vi "load vi modification tools.vi"() -> ()   [LabVIEW 2013, in "vi mod UI.lvlib"]
uses:
  vi mod UI.lvlib
  VI modification.lvclass
  collection/VI modification collection.lvclass
  collection/VI modification collection.lvclass/VI modification collection.ctl
  collection/Read current file list.vi
panel:
  in  "Report":i32(listbox)
  in  "Remove path":bool
  in  "add search":bool
  in  "Paths":i32(listbox)
  in  "run":bool
  in  "remove mod":bool
  in  "add mod":bool
  in  "Selected Tools":i32(listbox)
  in  "Available Tools":i32(listbox)
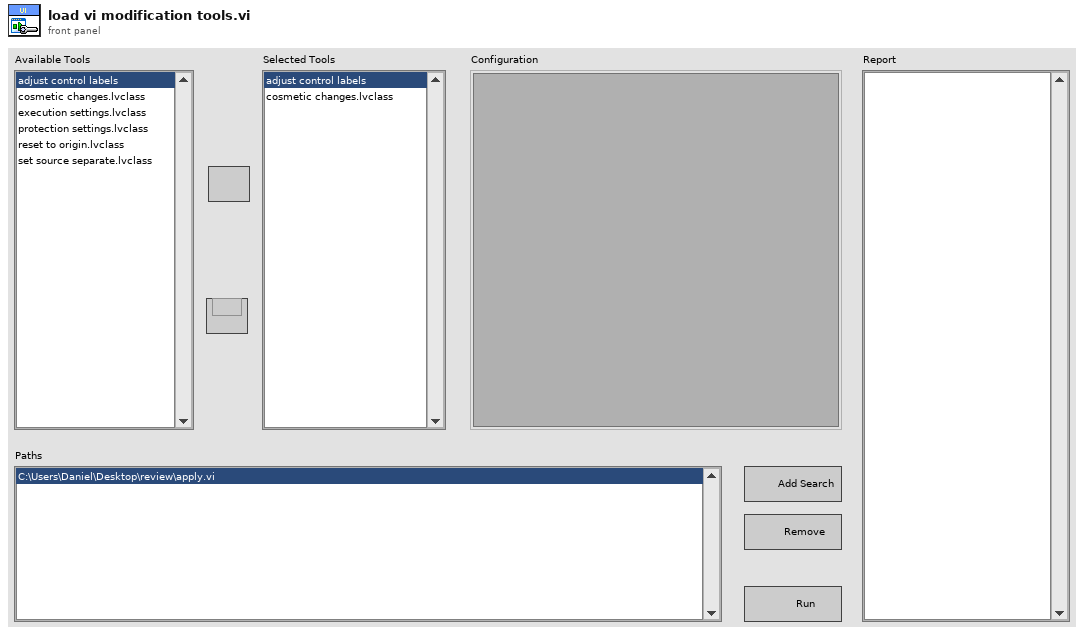
[diagram p1: front panel]
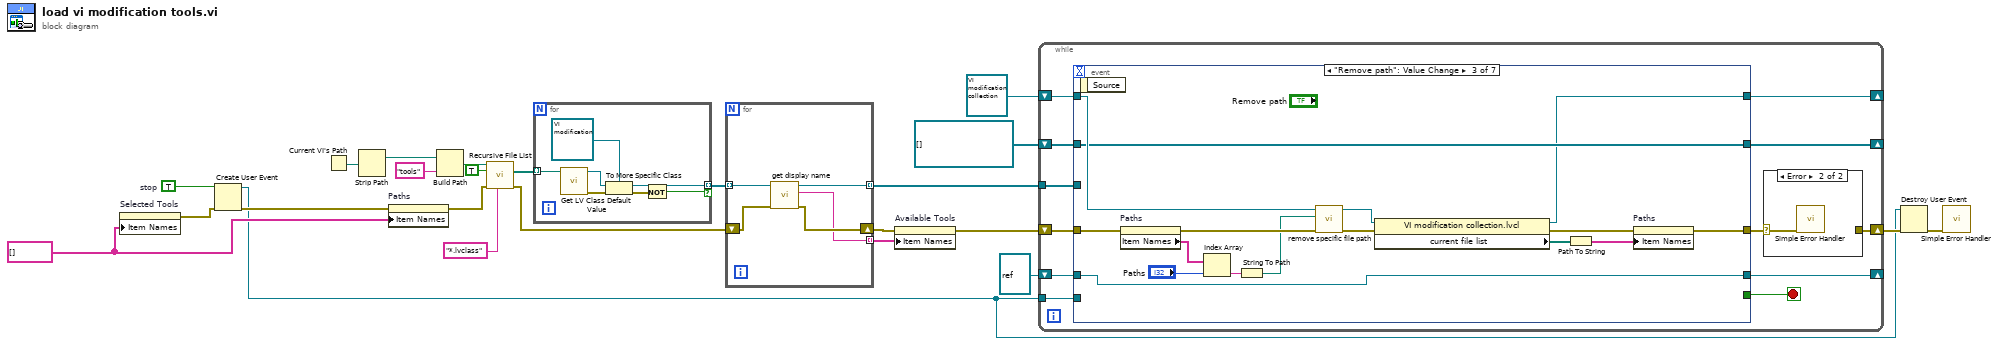
[diagram p0: block diagram]
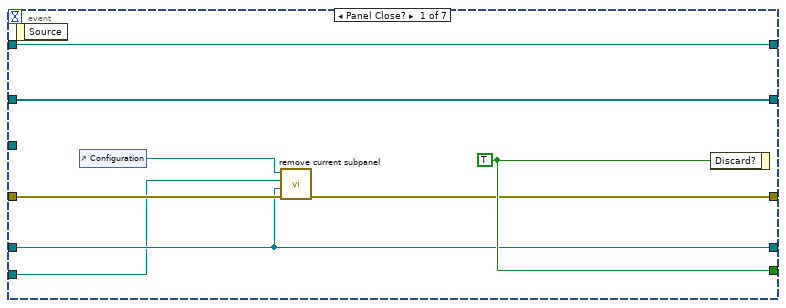
[diagram p3: hidden frame]
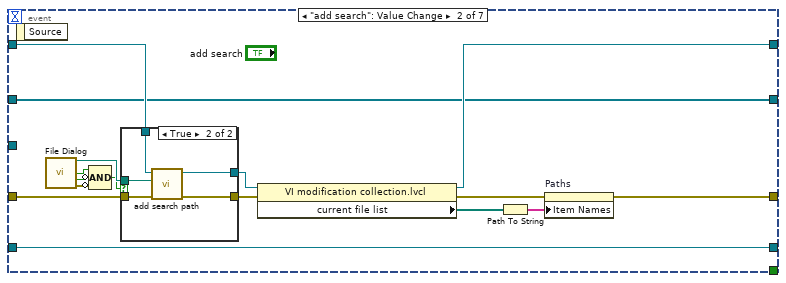
[diagram p4: hidden frame]
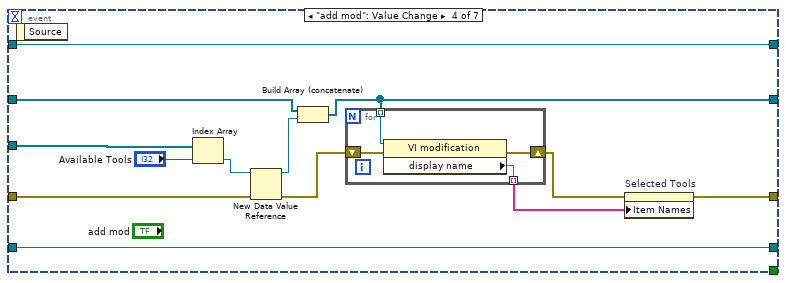
[diagram p6: hidden frame]
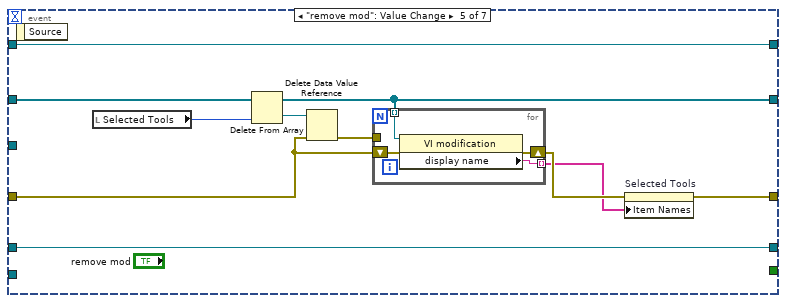
[diagram p7: hidden frame]
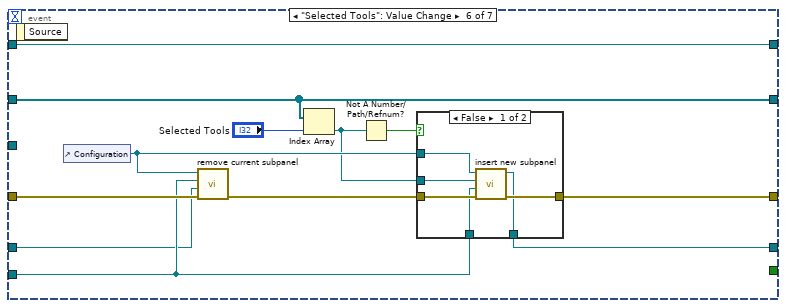
[diagram p8: hidden frame]
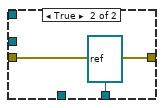
[diagram p9: hidden frame]
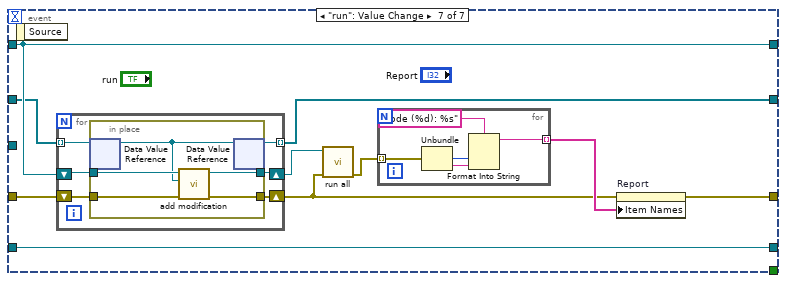
[diagram p10: hidden frame]
diagram:
  w7 = TRUE  # stop
  w5 = string[] [] ("Item Names")
  n1 = property on="Selected Tools" class="LstBox (strict)"("Item Names"=w5) -> (error out=w6:errorcluster)  [unwired: 2 in, 1 out]
  n2 = Create User Event(user event datatype=w7, error in=w6) -> (user event=w2:refnum<user-event>, error out=w8:errorcluster)
  n3 = Current VI's Path() -> (path=w24:path)
  n4 = Strip Path(path=w24) -> (stripped path=w23:path)  [unwired: 1 out]
  n5 = property on="Paths" class="LstBox (strict)"(error in=w8, "Item Names"=w5) -> (error out=w9:errorcluster)  [unwired: 1 in, 1 out]
  n6 = Build Path(base path=w23, name or relative path="tools") -> (appended path=w21:path)
  n7 = call <vilib>:"Recursive File List.vi"("pattern"="*.lvclass", "error in (no error)"=w9, "Treat LLBs as Folders?"=TRUE, "Folder Path"=w21) -> ("error out"=w16:errorcluster, "All Files in Dir"=w18:path[])  [unwired: 3 in, 3 out]
  n8 = for {
    tunnel: w18 -> [w31] mode=indexing
    tunnel: [w27] -> w17 mode=indexing if=w25
    n9 = call <vilib>:"Get LV Class Default Value.vi"("class path"=w31) -> ("error out"=w30:errorcluster, "object"=w29:refnum<class>)  [unwired: 9 in]
    n10 = To More Specific Class(target class=refnum<class "VI modification.lvclass"> refnum ("VI modification"), reference=w29, error in=w30) -> (specific class reference=w27:refnum<class "VI modification.lvclass">, error out=w26:errorcluster)
    n11 = Not(x=w26) -> (.not. x?=w25:bool)
  }
  n12 = for {
    tunnel: w17 -> [w36] mode=indexing
    shift-right: [w34] -> w15
    shift-left: w16 -> [w35]
    tunnel: [w33] -> w12 mode=indexing
    tunnel: [w32] -> w14 mode=indexing
    n13 = call-dynamic "get display name.vi"("error in"=w35, "VI modification in"=w36) -> ("error out"=w34:errorcluster, "class name"=w32:string, "VI modification out"=w33:refnum<class "VI modification.lvclass">)  [unwired: 7 in]
  }
  n14 = property on="Available Tools" class="LstBox (strict)"(error in=w15, "Item Names"=w14) -> (error out=w13:errorcluster)  [unwired: 1 in, 1 out]
  n15 = while {
    shift-right: [w39] -> w3
    shift-left: w13 -> [w48]
    tunnel: w12 -> [w46]
    shift-right: [w41] -> _
    shift-left: refnum<data-value>[] [] -> [w45]
    shift-right: [w43] -> _
    shift-left: refnum<class "VI modification collection.lvclass"> refnum ("VI modification collection.lvclass") -> [w44]
    tunnel: w2 -> [w42]
    shift-right: [w38] -> _
    shift-left: refnum<vi> refnum ("reference out") -> [w37]
    stop <- w47 stop-if-true
    n16 = event shown="[2] \"Remove path\": Value Change" {
      selector: _ -> [_ _ _ _ _ _ _]
      dyn-events: _ -> [_ _ _ _ _ _ _]
      timeout: _ -> [_ _ _ _ _ _ _]
      tunnel: w48 -> [w55 w74 w96 w104 w117 w140 w159]
      tunnel: [w54 w62 w82 w106 w124 w136 w154] -> w40
      tunnel: [w58 _ _ _ _ _ _] -> w47
      tunnel: w46 -> [_ _ _ w108 _ _ _]
      tunnel: w45 -> [w56 w60 w90 w109 w122 w139 w152]
      tunnel: [w56 w60 w90 w105 w121 w139 w151] -> w41
      tunnel: w44 -> [w57 w72 w97 w110 w125 w141 w158]
      tunnel: [w57 w65 w85 w110 w125 w141 w158] -> w43
      tunnel: w42 -> [w51 _ _ _ _ w134 _]
      tunnel: [w53 w59 w89 w98 w115 w130 w150] -> w38
      tunnel: w37 -> [w53 w59 w89 w98 w115 w131 w150]
      event Panel Close? {
        w58 = TRUE ("Discard?")
        n17 = event-data() -> ()  [unwired: 1 in, 1 out]
        n18 = control-ref of="Configuration"() -> (w52:refnum<vi>)
        n19 = call "remove current subpanel.vi"("error in"=w55, "current VI"=w53, "stop"=w51, "SubPanel in"=w52) -> ("error out"=w54:errorcluster)  [unwired: 7 in]
        n20 = event-data("Discard?"=w58) -> ()  [unwired: 1 in, 1 out]
      }
      event "add search": Value Change {
        n21 = event-data() -> ()  [unwired: 1 in, 1 out]
        n22 = call "File Dialog"() -> ("selected path"=w68:path, "exists"=w69:bool, "cancelled"=w70:bool, "error out"=w71:errorcluster)  [unwired: 12 in]
        n23 = Compound Arithmetic op=AND(w69, invert w70, invert w71) -> (w67:bool)
        n24 = case shown="True" w67 {
          tunnel: w74 -> [w75 w81]
          tunnel: [w75 w80] -> w73
          tunnel: w72 -> [w76 w79]
          tunnel: [w76 w78] -> w66
          tunnel: w68 -> [_ w77]
          frame False {
          }
          frame True {
            n25 = call "add search path.vi"("error in"=w81, "Path"=w77, "vi modification tool in"=w79) -> ("error out"=w80:errorcluster, "vi modification tool out"=w78:refnum<class "VI modification collection.lvclass">)  [unwired: 7 in]
          }
        }
        n26 = property class="VI modification collection.lvcl"(reference=w66, error in=w73) -> (reference out=w65:refnum<class "VI modification collection.lvclass">, error out=w63:errorcluster, "current file list"=w64:path[])
        n27 = Path To String(path=w64) -> (string=w61:string[])
        n28 = property on="Paths" class="LstBox (strict)"(error in=w63, "Item Names"=w61) -> (error out=w62:errorcluster)  [unwired: 1 in, 1 out]
      }
      event "Remove path": Value Change {
        n29 = event-data() -> ()  [unwired: 1 in, 1 out]
        n30 = property on="Paths" class="LstBox (strict)"(error in=w96) -> (error out=w95:errorcluster, "Item Names"=w94:string[])  [unwired: 1 in, 1 out]
        n31 = Index Array(array=w94, index="Paths") -> (element=w92:string)
        n32 = String To Path(string=w92) -> (path=w91:path)
        n33 = call "remove specific file path.vi"("error in"=w95, "Path"=w91, "VI modification collection in"=w97) -> ("error out"=w87:errorcluster, "VI modification collection out"=w86:refnum<class "VI modification collection.lvclass">)  [unwired: 7 in]
        n34 = property class="VI modification collection.lvcl"(reference=w86, error in=w87) -> (reference out=w85:refnum<class "VI modification collection.lvclass">, error out=w84:errorcluster, "current file list"=w88:path[])
        n35 = Path To String(path=w88) -> (string=w83:string[])
        n36 = property on="Paths" class="LstBox (strict)"(error in=w84, "Item Names"=w83) -> (error out=w82:errorcluster)  [unwired: 1 in, 1 out]
      }
      event "add mod": Value Change {
        n37 = event-data() -> ()  [unwired: 1 in, 1 out]
        n38 = Index Array(array=w108, index="Available Tools") -> (element=w101:refnum<class "VI modification.lvclass">)
        n39 = New Data Value Reference(data value=w101, error in=w104) -> (data value reference=w100:refnum<data-value>, error out=w102:errorcluster)
        n40 = Build Array (concatenate)(w109, w100) -> (w105:refnum<data-value>[])
        n41 = for {
          tunnel: w105 -> [w113] mode=indexing
          shift-right: [w112] -> w103
          shift-left: w102 -> [w114]
          tunnel: [w111] -> w99 mode=indexing
          n42 = property class="VI modification"(reference=w113, error in=w114) -> (error out=w112:errorcluster, "display name"=w111:string)  [unwired: 1 out]
        }
        n43 = property on="Selected Tools" class="LstBox (strict)"(error in=w103, "Item Names"=w99) -> (error out=w106:errorcluster)  [unwired: 1 in, 1 out]
      }
      event "remove mod": Value Change {
        n44 = event-data() -> ()  [unwired: 1 in, 1 out]
        n45 = local read "Selected Tools"() -> (w120:i32)
        n46 = Delete From Array(array=w122, index=w120) -> (deleted portion=w118:refnum<data-value>, array with subset deleted=w121:refnum<data-value>[])  [unwired: 1 in]
        n47 = Delete Data Value Reference(data value reference=w118, error in=w117) -> (error out=w116:errorcluster)  [unwired: 1 out]
        n48 = for {
          tunnel: w121 -> [w127] mode=indexing
          shift-right: [w129] -> w123
          shift-left: w117 -> [w128]
          tunnel: [w126] -> w119 mode=indexing
          tunnel: w116 -> [_]
          n49 = property class="VI modification"(reference=w127, error in=w128) -> (error out=w129:errorcluster, "display name"=w126:string)  [unwired: 1 out]
        }
        n50 = property on="Selected Tools" class="LstBox (strict)"(error in=w123, "Item Names"=w119) -> (error out=w124:errorcluster)  [unwired: 1 in, 1 out]
      }
      event "Selected Tools": Value Change {
        n51 = event-data() -> ()  [unwired: 1 in, 1 out]
        n52 = control-ref of="Configuration"() -> (w135:refnum<vi>)
        n53 = call "remove current subpanel.vi"("error in"=w140, "current VI"=w131, "stop"=w134, "SubPanel in"=w135) -> ("error out"=w137:errorcluster)  [unwired: 7 in]
        n54 = Index Array(array=w139, index="Selected Tools") -> (element=w133:refnum<data-value>)
        n55 = Not A Number/Path/Refnum?(number/path/refnum=w133) -> (NaN/Path/Refnum?=w132:bool)
        n56 = case shown="False" w132 {
          tunnel: w137 -> [w147 w149]
          tunnel: [w146 w149] -> w136
          tunnel: w135 -> [w145 _]
          tunnel: w134 -> [w144 _]
          tunnel: w133 -> [w143 _]
          tunnel: [w142 refnum<vi> refnum ("reference out")] -> w130
          frame False {
            n57 = call "insert new subpanel.vi"("error in"=w147, "event"=w144, "mod data ref"=w143, "SubPanel in"=w145) -> ("error out"=w146:errorcluster, "reference out"=w142:refnum<vi>)  [unwired: 6 in]
          }
          frame True {
          }
        }
      }
      event "run": Value Change {
        n58 = event-data() -> ()  [unwired: 1 in, 1 out]
        n59 = for {
          shift-right: [w167] -> w153
          shift-left: w159 -> [w170]
          shift-right: [w168] -> w157
          shift-left: w158 -> [w169]
          tunnel: w152 -> [w166] mode=indexing
          tunnel: [w165] -> w151 mode=indexing
          n60 = in-place {
            in-place-border: w170 -> [w175]
            in-place-border: w169 -> [w174]
            in-place-border: [w173] -> w168
            in-place-border: [w172] -> w167
            n61 = in-place-dvr #1(w166) -> (w171:refnum<class "VI modification.lvclass">)  [unwired: 1 out]
            n62 = call "add modification.vi"("error in"=w175, "VI modification"=w171, "vi modification tool in"=w174) -> ("error out"=w172:errorcluster, "vi modification tool out"=w173:refnum<class "VI modification collection.lvclass">)  [unwired: 7 in]
            n63 = in-place-dvr #1(w171) -> (w165:refnum<data-value>)  [unwired: 1 out]
          }
        }
        n64 = call "run all.vi"("error in"=w153, "vi modification tool in"=w157) -> ("error report"=w156:errorcluster[])  [unwired: 8 in, 1 out]
        n65 = for {
          tunnel: w156 -> [w164] mode=indexing
          tunnel: [w160] -> w155 mode=indexing
          n66 = Unbundle(w164) -> ("code"=w163:i32, "source"=w162:string)  [unwired: 1 out]
          n67 = Format Into String(format string="code (%d): %s", w163, w162) -> (resulting string=w160:string)  [unwired: 2 in, 1 out]
        }
        n68 = property on="Report" class="LstBox (strict)"(error in=w153, "Item Names"=w155) -> (error out=w154:errorcluster)  [unwired: 1 in, 1 out]
      }
    }
    n69 = case shown="Error" w40 {
      selector: w40 -> [w49 w50]
      tunnel: [w49 _] -> w39
      frame No Error {
      }
      frame Error {
        n70 = call <vilib>:"Simple Error Handler.vi"("error in (no error)"=w50) -> ()  [unwired: 4 in, 5 out]
      }
    }
  }
  n71 = Destroy User Event(user event=w2, error in=w3) -> (error out=w1:errorcluster)
  n72 = call <vilib>:"Simple Error Handler.vi"("error in (no error)"=w1) -> ()  [unwired: 4 in, 5 out]
